vi "Run Test (ProjectRefnum).vi"(4 "timeout (2000 ms)":i32=2000, 5 "Test Report":refnum<class "Test Report.lvclass">, 6 "Verbose":bool, 7 "Report Path":path, 8 "error in":errorcluster, 9 "Virtual Folder (My Computer)":string, 10 "Project Refnum":refnum<vi>, 11 "Interactive (T)":bool=TRUE) -> (0 "error out":errorcluster, 3 "Test Results":refnum<class "Test Result.lvclass">)   [LabVIEW 2020, in "Caraya.lvlib"]
doc: "\"Run Tests\" from a preject reference:\n- Dynamically discovers Caraya unit tests and runs them\n- Outputs results in a UI ans/or Test Report (J-Unit or text)\n\n(Not compatible with RT targets or RunTime Engine)"
uses:
  Caraya.lvlib
  classes/Test Report/Test Report.lvclass
  classes/Test Result/Test Result.lvclass
  classes/Test Runner.Project/Test Runner.Project.lvclass
  C:/projects/caraya/src/classes/Test Runner/Test Runner.lvclass
  classes/Test Runner/Test Runner.lvclass
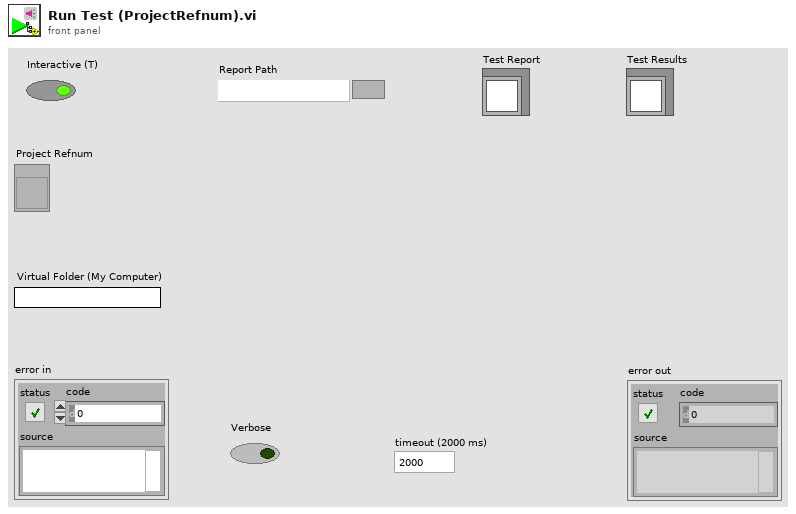
[diagram p1: front panel]
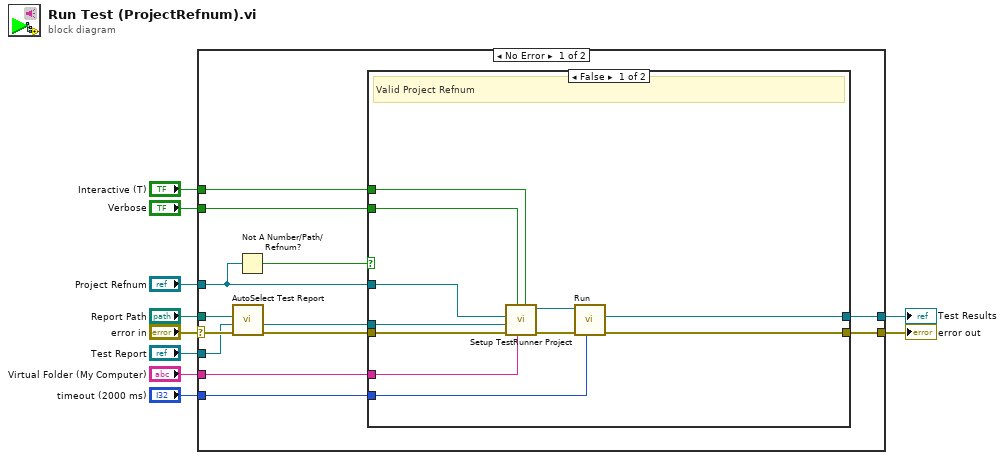
[diagram p0: block diagram]
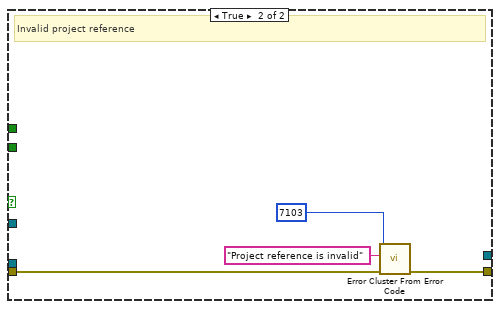
[diagram p2: hidden frame]
diagram:
  n1 = case shown="No Error" "error in" {
    selector: "error in" -> [w20 w39]
    tunnel: [w23 w39] -> w10
    tunnel: "Verbose" -> [w22 _]
    tunnel: "Interactive (T)" -> [w21 _]
    tunnel: "Test Report" -> [w17 _]
    tunnel: "Project Refnum" -> [w14 _]
    tunnel: "Report Path" -> [w19 _]
    tunnel: "Virtual Folder (My Computer)" -> [w15 _]
    tunnel: "timeout (2000 ms)" -> [w12 _]
    tunnel: [w11 _] -> w1
    frame No Error {
      n2 = call "AutoSelect Test Report.vi"("error in (no error)"=w20, "Test Report in"=w17, "Report Path"=w19) -> ("error out"=w18:errorcluster, "Test Report out"=w16:refnum<class "Test Report.lvclass">)  [unwired: 7 in]
      n3 = Not A Number/Path/Refnum?(number/path/refnum=w14) -> (NaN/Path/Refnum?=w13:bool)
      n4 = case shown="False" w13 {
        tunnel: [w34 w37] -> w23
        tunnel: w22 -> [w33 _]
        tunnel: w21 -> [w32 _]
        tunnel: w18 -> [w29 w38]
        tunnel: w16 -> [w28 _]
        tunnel: w15 -> [w27 _]
        tunnel: w14 -> [w26 _]
        tunnel: w12 -> [w25 _]
        tunnel: [w24 _] -> w11
        frame False {
          # "Valid Project Refnum"
          n5 = call "Setup TestRunner Project.vi"("Interactive (T)"=w32, "Virtual Folder (empty: \"My Computer\")"=w27, "Verbose (F)"=w33, "error in (no error)"=w29, "Test Report"=w28, "Project Refnum"=w26) -> ("error out"=w30:errorcluster, "Test Runner.Project out"=w31:refnum<class "Test Runner.Project.lvclass">)  [unwired: 4 in]
          n6 = call "Run.vi"("timeout"=w25, "error in (no error)"=w30, "Test Runner in"=w31) -> ("error out"=w34:errorcluster, "Test Suite Results"=w24:refnum<class "Test Result.lvclass">)  [unwired: 6 in, 1 out]
        }
        frame True {
          # "Invalid project reference"
          n7 = call <vilib>:"Error Cluster From Error Code.vi"("error in (no error)"=w38, "error message (\"\")"="Project reference is invalid" ("error message (\"\")"), "error code (0)"=7103 ("code")) -> ("error out"=w37:errorcluster)  [unwired: 6 in]
        }
      }
    }
    frame Error {
    }
  }
  "error out" <- w10
  "Test Results" <- w1
